vi "zadanie_1_lab0.vi"(10 "Zmienna  2":dbl, 11 "Zmienna 1":dbl) -> ()   [LabVIEW 2020]
panel:
  out "Czy zmienna 3 jest mniejsza b¹d¿ równa sumie zmiennej 1 oraz zmiennej 2?":bool
  out "iloczyn zmiennej 1 oraz 2":dbl
  out "Czy iloczyn zmiennej 1 oraz 2 nie jest równy zmiennej 3 ?":bool
  out "ró¿nica  zmiennej 1 oraz 2":dbl
  in  "Zmienna 3":dbl
  out "Czy zmienna 3 jest wiêksza od ró¿nicy zmiennej 1 oraz zmiennej 2 ?":bool
  out "suma zmiennej 1 oraz 2":dbl
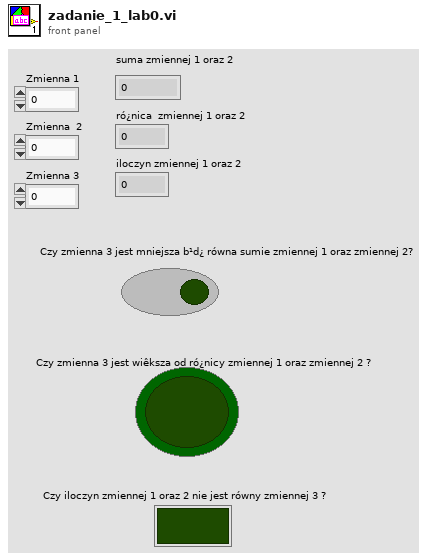
[diagram p1: front panel]
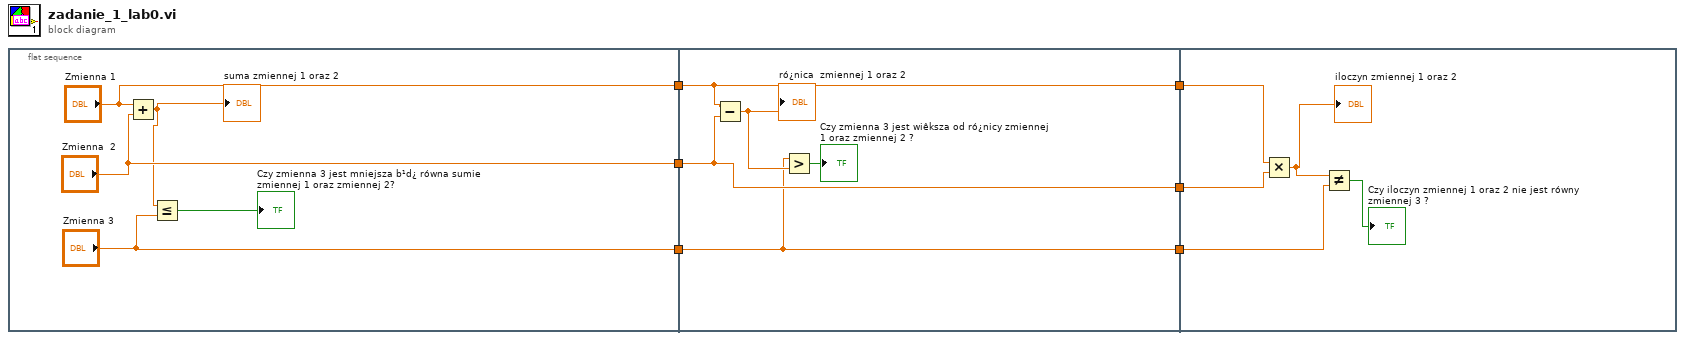
[diagram p0: block diagram]
diagram:
  n1 = flat-sequence {
    tunnel: ["Zmienna  2"] -> w6
    tunnel: ["Zmienna 1"] -> w5
    tunnel: ["Zmienna 3"] -> w4
    tunnel: w6 -> [w13]
    tunnel: w5 -> [w14]
    tunnel: w4 -> [w12]
    tunnel: [w14] -> w3
    tunnel: [w13] -> w2
    tunnel: [w12] -> w1
    tunnel: w3 -> [w21]
    tunnel: w2 -> [w20]
    tunnel: w1 -> [w19]
    frame #0 {
      n2 = Add(x="Zmienna 1", y="Zmienna  2") -> (x+y=w9:dbl)
      "suma zmiennej 1 oraz 2" <- w9
      n3 = Less Or Equal?(x=w9, y="Zmienna 3") -> (x <= y?=→"Czy zmienna 3 jest mniejsza b¹d¿ równa sumie zmiennej 1 oraz zmiennej 2?":bool)
    }
    frame #1 {
      n4 = Subtract(x=w14, y=w13) -> (x-y=w15:dbl)
      "ró¿nica  zmiennej 1 oraz 2" <- w15
      n5 = Greater?(x=w12, y=w15) -> (0:→"Czy zmienna 3 jest wiêksza od ró¿nicy zmiennej 1 oraz zmiennej 2 ?":bool)
    }
    frame #2 {
      n6 = Multiply(x=w21, y=w20) -> (x*y=w17:dbl)
      "iloczyn zmiennej 1 oraz 2" <- w17
      n7 = Not Equal?(x=w17, y=w19) -> (x != y?=→"Czy iloczyn zmiennej 1 oraz 2 nie jest równy zmiennej 3 ?":bool)
    }
  }
